vi "PhotonCamera_IsConnected.vi"(8 "Pass_Through_Time":dbl=-1.0 format="%33.4f", 9 "BaseNTName":string="/photonvision", 11 "CameraName":string) -> (0 "error out":errorcluster, 3 "IsConnected":bool)   [LabVIEW 2019, in "PhotonVisionLib.lvlib"]
doc: "Determines if communications to camera is valid.\n\nInputs:\n - CameraName -- The nickname of the camera (found in the PhotonVision UI).\n - BaseNTName - string - Base Nework Table name. (Optional. Default: /photonvision )\n \nOutputs:\n - IsConnected -- TRUE if communications have been received within the last 0.5 seconds.\n - Error Out -- Contains error information if a Network table ot other error occured."
uses:
  PhotonVisionLib.lvlib
  <vilib>/Rock Robotics/WPI/ThirdParty/JAS_Junk/TrajLib/VI/Util_GetTime_U32.vi
  <vilib>/Rock Robotics/WPI/ThirdParty/JAS_Junk/TrajLib/VI/Util_GetTime_U64.vi
  <vilib>/Rock Robotics/Network Tables/NT Read Integer.vi
  <vilib>/Rock Robotics/WPI/ThirdParty/JAS_Junk/TrajLib/Trajectory_Library.lvlib
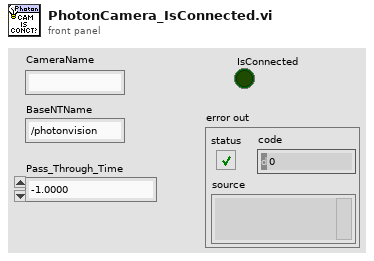
[diagram p1: front panel]
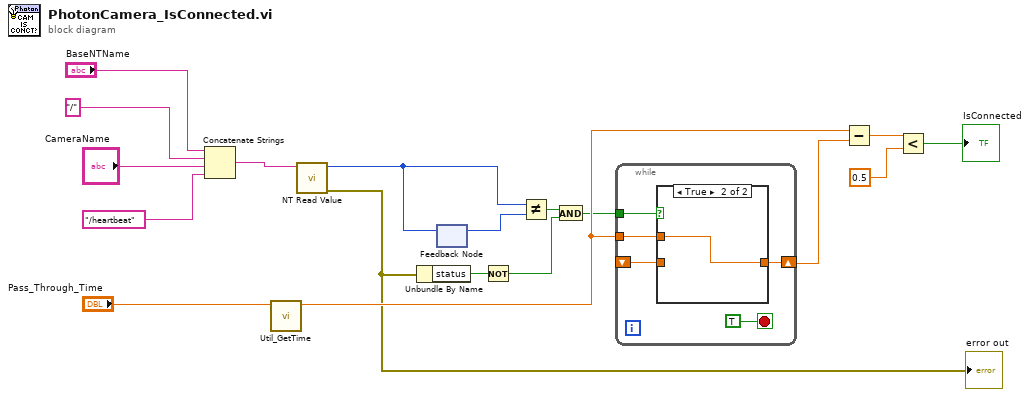
[diagram p0: block diagram]
diagram:
  n1 = Concatenate Strings("BaseNTName", "/", "CameraName", "/heartbeat") -> (w15:string)
  n2 = call <vilib>:"Util_GetTime.vi"("Pass_Through_Time"="Pass_Through_Time") -> ("FPGA_Time_Seconds"=w11:dbl)  [unwired: 8 in, 2 out]
  n3 = call-poly <vilib>:"NT Read Value.vi"("name"=w15) -> ("error out"=w5:errorcluster, "value"=w12:i64)  [unwired: 8 in, 1 out]
  "error out" <- w5
  n4 = Unbundle By Name(w5) -> ("status"=w3:bool)
  n5 = feedback-in #1(w12) -> ()
  n6 = feedback #1() -> (w13:i64)  [unwired: 1 in]
  n7 = Not(x=w3) -> (.not. x?=w2:bool)
  n8 = Not Equal?(x=w12, y=w13) -> (x != y?=w6:bool)
  n9 = And(x=w6, y=w2) -> (x .and. y?=w4:bool)
  n10 = while {
    tunnel: w4 -> [w22]
    tunnel: w11 -> [w21]
    shift-right: [w20] -> w10
    shift-left: _ -> [w19]
    stop <- TRUE stop-if-true
    n11 = case shown="True" w22 {
      tunnel: [w24 w25] -> w20
      tunnel: w21 -> [_ w25]
      tunnel: w19 -> [w24 _]
      frame False {
      }
      frame True {
      }
    }
  }
  n12 = Subtract(x=w11, y=w10) -> (x-y=w9:dbl)
  n13 = Less?(x=w9, y=0.5) -> (x < y?=→"IsConnected":bool)
